vi "init Sweep Measurement.vi"(8 "error in (no error)":errorcluster, 10 "Sweep Measurement Mode":enum16{"Single Sweep", "Continuous Sweep"}(ring), 11 "FSV-40N in":refnum<class "FSV-40N.lvclass">) -> (0 "error out":errorcluster, 3 "FSV-40N out":refnum<class "FSV-40N.lvclass">)   [LabVIEW 2023, in "Spectrum Analyzer.lvlib" / "FSV-40N.lvclass"]
uses:
  FSV-40N.lvclass
  FSV-40N.lvclass/FSV-40N.ctl
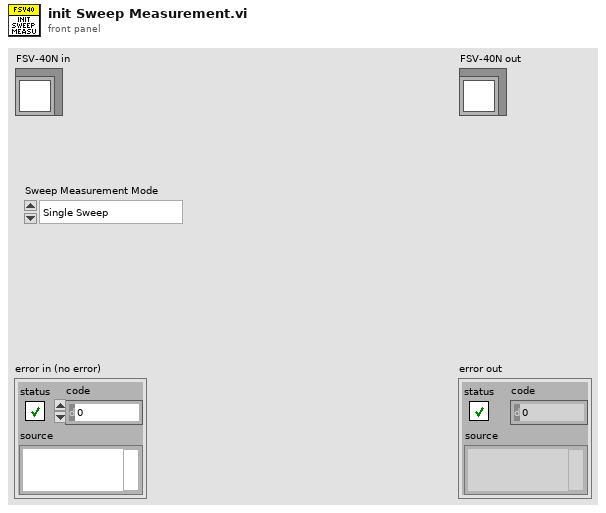
[diagram p1: front panel]
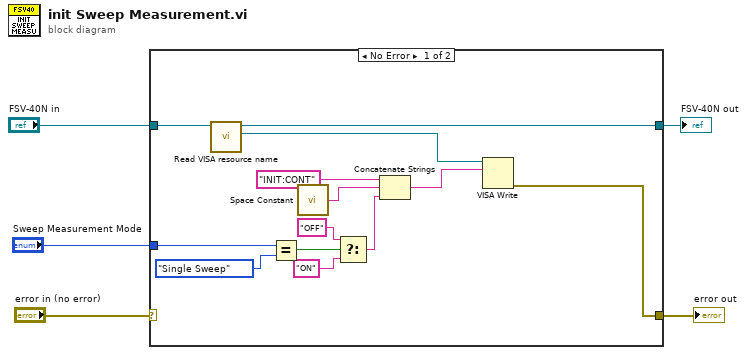
[diagram p0: block diagram]
diagram:
  n1 = case shown="No Error" "error in (no error)" {
    selector: "error in (no error)" -> [_ w20]
    tunnel: "FSV-40N in" -> [w18 w19]
    tunnel: [w7 w20] -> w3
    tunnel: [w6 w19] -> w2
    tunnel: "Sweep Measurement Mode" -> [w15 _]
    frame No Error {
      n2 = call "Read VISA resource name.vi"("FSV-40N in"=w18) -> ("VISA resource name"=w9:refnum<visa-resource-name>, "FSV-40N out"=w6:refnum<class "FSV-40N.lvclass">)  [unwired: 8 in, 1 out]
      n3 = Equal?(x=w15, y=enum16{"Single Sweep", "Continuous Sweep"}."Single Sweep") -> (x = y?=w13:bool)
      n4 = call <vilib>:"Space Constant.vi"() -> ("String"=w16:string)
      n5 = Select(t="OFF", s=w13, f="ON") -> (s? t:f=w10:string)
      n6 = Concatenate Strings("INIT:CONT" ("string"), w16, w10) -> (w8:string)
      n7 = VISA Write(VISA resource name=w9, write buffer=w8) -> (error out=w7:errorcluster)  [unwired: 1 in, 2 out]
    }
    frame Error {
    }
  }
  "error out" <- w3
  "FSV-40N out" <- w2
